vi "Channel Read Write.vi"(11 "plugin gRPC address":string="localhost:51930") -> ()   [LabVIEW 2021, in "CAN_Writer_CANsub_Test_Helpers.lvlib"]
uses:
  CAN_Writer_CANsub_Test_Helpers.lvlib
  <vilib>/CIF Foundation/CIF Core/CIFCore/Grpc/CIFCoreWrapper/CIFCoreWrapper.lvlib
  <vilib>/CIF Foundation/CIF Core/CIFCore/Class/CIFCorePlugin.lvclass
  Common/Typedef/Channels.ctl
  Common/CAN_Writer_CANsub_Common.lvlib
  Grpc/CAN_Writer_CANsub_wrapper/CAN_Writer_CANsub_Wrapper.lvlib
  <vilib>/CIF Foundation/CIF Channels Core/ChannelCommon/typedef/TimeStamps.ctl
  <vilib>/CIF Foundation/CIF Channels Core/ChannelCommon/ChannelCommon.lvlib
  <vilib>/CIF Foundation/CIF Utilities/Time/Time_CIF_U.lvlib
  <vilib>/CIF Foundation/CIF XNET CAN RW/XNET CAN RW.lvclass
  <vilib>/CIF Foundation/CIF Core/CIFCore/Common/Typedef/Plugin State.ctl
  <vilib>/CIF Foundation/CIF Core/CIFCore/Common/CIFCoreCommon.lvlib
  <vilib>/CIF Foundation/CIF Core/CIFCore/Common/Typedef/Timing Stats Base.ctl
  <vilib>/CIF Foundation/CIF Core/CIFCore/Common/Typedef/Timing Statistics.ctl
  <vilib>/CIF Foundation/CIF Core/CIFCore/Common/Typedef/FIFO Statistics.ctl
  <vilib>/CIF Foundation/CIF Core/CIFCore/Common/Typedef/Simple Error.ctl
  <vilib>/CIF Foundation/CIF Core/CIFCore/Common/Typedef/Monitor Doubles.ctl
  <vilib>/CIF Foundation/CIF Core/CIFCore/Common/Typedef/Monitor U64.ctl
  <vilib>/CIF Foundation/CIF Core/CIFCore/Common/Typedef/Monitor I64.ctl
  <vilib>/CIF Foundation/CIF Core/CIFCore/Common/Typedef/gRPC Reported Plugin Status.ctl
  <vilib>/xnet/xnet.llb/XNET Frame Type CAN.ctl
  <vilib>/xnet/xnet.llb/XNET Frame CAN.ctl
panel:
  in  "CAN Data":T1[](array[typedef])=[{"timestamp"=timestamp(3831573600 s since 1904-01-01), "payload"=[1, 2, 3, 4, 5, 6, 7, 8], "identifier"=33, "type"=16, "extended?"=TRUE, "echo?"=FALSE}, {"timestamp"=timestamp(3831570000 s since 1904-01-01), "payload"=[10, 11, 10, 13, 11, 10, 11, 14], "identifier"=82, "type"=0, "extended?"=TRUE, "echo?"=FALSE}] {"payload" format="%x"; "timestamp" format="%<%.7X\n%x>T"; "type" items=["CAN Data"=0, "CAN Remote"=1, "CAN Bus Error"=2, "CAN 2.0 Data"=8, "CAN FD Data"=16, "CAN FD+BRS Data"=24, "J1939 Data"=192, "Delay"=224, "Log Trigger"=225, "Start Trigger"=226]; "identifier" format="%x"}
  in  "Offset (ns)":i64=1000000000 format="%.0e"
  out "Node Status":T3 {"Monitor Doubles"."4" format="%#_9g"; "Monitor Doubles"."3" format="%#_9g"; "Monitor Doubles"."2" format="%#_9g"; "Monitor Doubles"."1" format="%#_9g"; "Timing Statistics (us)"."Period"."Avg" format="%_6g"}
  in  "EXIT":bool
  in  "Unload":bool
  out "error out":errorcluster
  # "Update plugin gRPC address including gRPC port and run on same target as the plugin code. \nExit will stop this VI.\nUnload will stop this VI and unload the plugin."
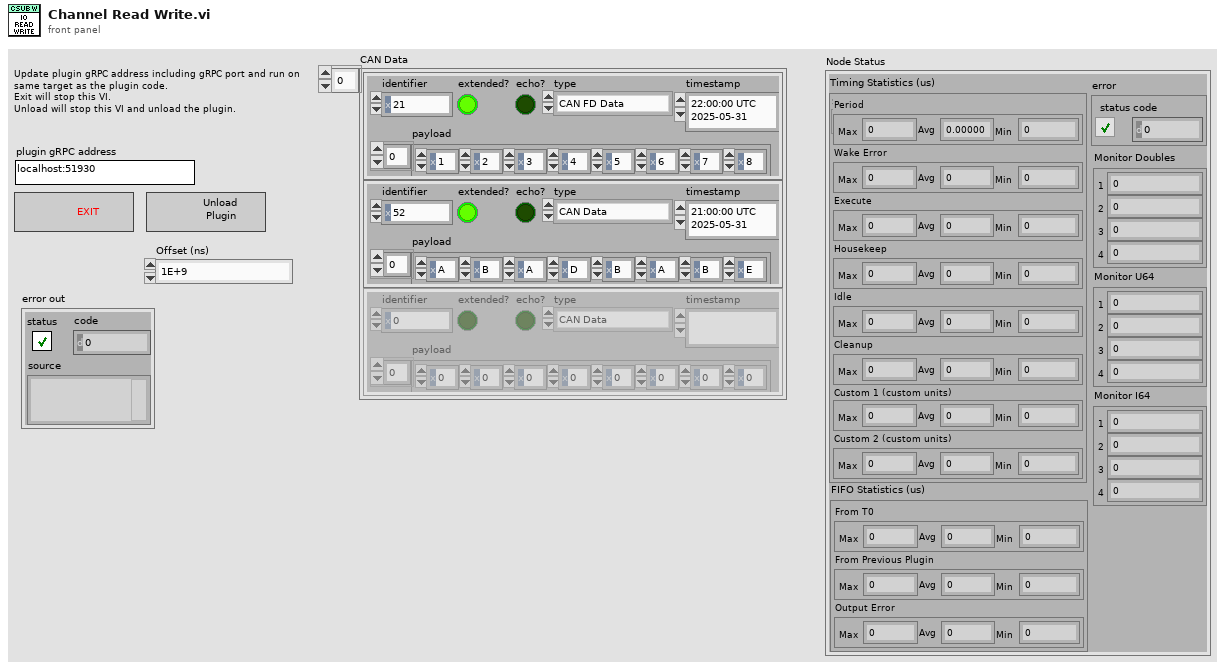
[diagram p1: front panel]
types:
  T1 = typedef "XNET Frame CAN.ctl" = cluster{"timestamp":timestamp, "payload":u8[], "identifier":u32, "type":T2, "extended?":bool, "echo?":bool}
  T2 = typedef "XNET Frame Type CAN.ctl" = u8
  T3 = typedef "CIFCoreCommon.lvlib/gRPC Reported Plugin Status.ctl" = cluster{"State":T4, "Timing Statistics (us)":T5, "FIFO Statistics (us)":T7, "error":T8, "Monitor Doubles":T9, "Monitor U64":T10, "Monitor I64":T11}
  T4 = typedef "CIFCoreCommon.lvlib/Plugin State.ctl" = enum8{"Null", "Creating", "Listening", "Running", "CleaningUp", "Destroying", "Prepared", "FTE_Run"}
  T5 = typedef "CIFCoreCommon.lvlib/Timing Statistics.ctl" = cluster{"Period":T6, "Wake Error":T6, "Execute":T6, "Housekeep":T6, "Idle":T6, "Cleanup":T6, "Custom 1 (custom units)":T6, "Custom 2 (custom units)":T6}
  T6 = typedef "CIFCoreCommon.lvlib/Timing Stats Base.ctl" = cluster{"Max":i64, "Avg":dbl, "Min":i64}
  T7 = typedef "CIFCoreCommon.lvlib/FIFO Statistics.ctl" = cluster{"From T0":T6, "From Previous Plugin":T6, "Output Error":T6}
  T8 = typedef "CIFCoreCommon.lvlib/Simple Error.ctl" = cluster{"status":bool, "code":i32}
  T9 = typedef "CIFCoreCommon.lvlib/Monitor Doubles.ctl" = cluster{"1":dbl, "2":dbl, "3":dbl, "4":dbl}
  T10 = typedef "CIFCoreCommon.lvlib/Monitor U64.ctl" = cluster{"1":u64, "2":u64, "3":u64, "4":u64}
  T11 = typedef "CIFCoreCommon.lvlib/Monitor I64.ctl" = cluster{"1":i64, "2":i64, "3":i64, "4":i64}
  T12 = typedef "grpc-lvsupport-release.lvlib/grpcId.ctl" = u64
  T13 = typedef "CIFCoreChannel_client.lvlib/cif_management_common_Channel.ctl" = cluster{"name":string, "direction":T14, "type":string, "custom_config":u8[], "connected":bool, "connected_name":string, "forced":bool, "channel_pattern":T15}
  T14 = typedef "CIFCoreChannel_client.lvlib/cif_management_common_ChannelDirection.ctl" = enum32{"CHANNELDIRECTION_UNKNOWN", "CHANNELDIRECTION_PUBLISHER", "CHANNELDIRECTION_SUBSCRIBER"}
  T15 = typedef "CIFCoreChannel_client.lvlib/cif_management_common_ChannelPattern.ctl" = enum32{"CHANNELPATTERN_UNKNOWN", "CHANNELPATTERN_TAG", "CHANNELPATTERN_FIFO", "CHANNELPATTERN_MULTIFIFO", "CHANNELPATTERN_BACKPRESSUREFIFO"}
  T16 = typedef "ChannelCommon.lvlib/TimeStamps.ctl" = cluster{"ClockID":u8, "T0":i64, "T_Out":i64}
  T17 = typedef "CAN_Writer_CANsub_Common.lvlib/Channels.ctl" = enum16{"CAN_Frames"}
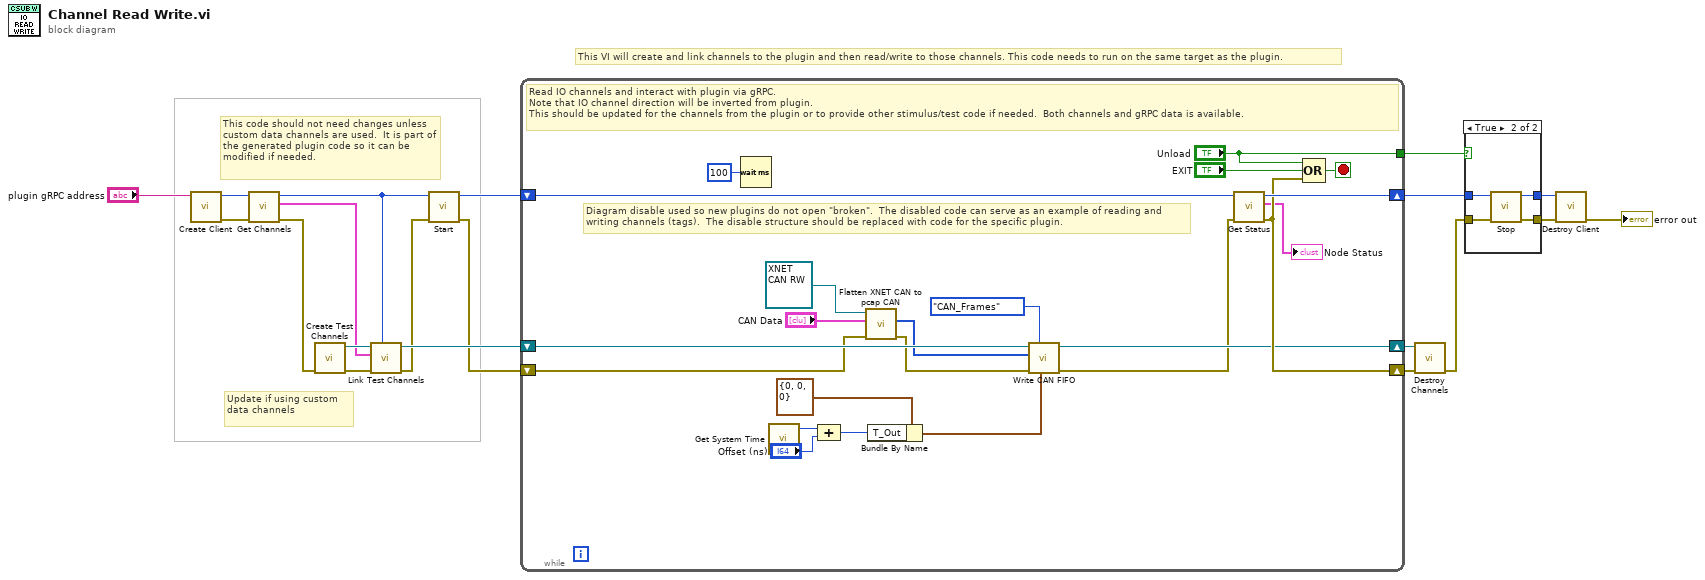
[diagram p0: block diagram]
diagram:
  # "Update if using custom data channels"
  # "This code should not need changes unless custom data channels are used.  It is part of the generated plugin code so it can be modified if needed."
  # "This VI will create and link channels to the plugin and then read/write to those channels. This code needs to run on the same target as the plugin."
  n1 = call "Create Client.vi"("address"="plugin gRPC address") -> ("error out"=w11:errorcluster, "gRPC ID Out"=w10:T12)  [unwired: 9 in]
  n2 = call <vilib>:"Get Channels.vi"("error in"=w11, "gRPC ID"=w10) -> ("error out"=w19:errorcluster, "Channels"=w15:T13[], "gRPC ID out"=w9:T12)  [unwired: 7 in]
  n3 = call "Create Test Channels.vi"("error in"=w19) -> ("error out"=w18:errorcluster, "CIFCorePlugin out"=w17:refnum<class "CIFCorePlugin.lvclass">)  [unwired: 9 in]
  n4 = call "Link Test Channels.vi"("gRPC ID in"=w9, "error in (no error)"=w18, "Channels"=w15, "CIFCorePlugin in"=w17) -> ("error out"=w7:errorcluster, "CIFCorePlugin out"=w16:refnum<class "CIFCorePlugin.lvclass">)  [unwired: 6 in]
  n5 = call <vilib>:"Start.vi"("error in"=w7, "gRPC ID"=w9) -> ("error out"=w6:errorcluster, "gRPC ID out"=w8:T12)  [unwired: 8 in]
  n6 = while {
    shift-right: [w33] -> w20
    shift-left: w16 -> [w34]
    shift-right: [w39] -> w14
    shift-left: w6 -> [w23]
    shift-right: [w41] -> w4
    shift-left: w8 -> [w42]
    tunnel: ["Unload"] -> w1
    stop <- w38 stop-if-true
    # "Diagram disable used so new plugins do not open \"broken\".  The disabled code can serve as an example of reading and writing channels (tags).  The disable structure should be replaced with code for the specific plugin."
    # "Read IO channels and interact with plugin via gRPC.\nNote that IO channel direction will be inverted from plugin.\nThis should be updated for the channels from the plugin or to provide other stimulus/test code if needed.  Both channels and gRPC data is available."
    n7 = Wait (ms)(milliseconds to wait=u32 100) -> ()  [unwired: 1 out]
    n8 = call <vilib>:"Get System Time.vi"() -> ("Time (ns)"=w29:i64)  [unwired: 5 in]
    n9 = Compound Arithmetic op=ADD(w29, "Offset (ns)") -> (w28:i64)
    n10 = call <vilib>:"Flatten XNET CAN to pcap CAN.vi"("error in (no error)"=w23, "XNET CAN Data"="CAN Data", "XNET_CAN_RW in"=refnum<class "XNET CAN RW.lvclass"> refnum ("CAN_Logic in")) -> ("error out"=w22:errorcluster, "pcap CAN DATA"=w21:u8[])  [unwired: 6 in, 1 out]
    n11 = Bundle By Name(cluster=T16 {"ClockID"=0, "T0"=0, "T_Out"=0} ("FIFO Timestamps"), "T_Out"=w28) -> (w26:T16)
    n12 = call <vilib>:"Write CAN FIFO.vi"("FIFO Timestamps"=w26, "Channel Index"=Channels."CAN_Frames" ("Channels"), "error in (no error)"=w22, "Data"=w21, "CIFCorePlugin in"=w34) -> ("error out"=w32:errorcluster, "CIFCorePlugin out"=w33:refnum<class "CIFCorePlugin.lvclass">)  [unwired: 4 in, 1 out]
    n13 = call <vilib>:"Get Status.vi"("error in"=w32, "gRPC ID"=w42) -> ("error out"=w39:errorcluster, "Node Status"=→"Node Status":T3, "gRPC ID out"=w41:T12)  [unwired: 7 in]
    n14 = Compound Arithmetic op=OR("Unload", "EXIT", w39) -> (w38:bool)
  }
  n15 = call <vilib>:"Destroy Channels.vi"("error in (no error)"=w14, "CIFCorePlugin in"=w20) -> ("error out"=w5:errorcluster)  [unwired: 7 in, 2 out]
  n16 = case shown="True" w1 {
    tunnel: w5 -> [w43 w48]
    tunnel: w4 -> [w44 w47]
    tunnel: [w44 w46] -> w3
    tunnel: [w43 w45] -> w2
    frame False {
    }
    frame True {
      n17 = call <vilib>:"Stop.vi"("error in"=w48, "gRPC ID"=w47) -> ("error out"=w45:errorcluster, "gRPC ID out"=w46:T12)  [unwired: 8 in]
    }
  }
  n18 = call "Destroy Client.vi"("error in"=w2, "gRPC ID"=w3) -> ("error out"=→"error out":errorcluster)  [unwired: 9 in]
